vi "UnscentedKalmanFilter_Correct_FuncGroup.vi"(0 "addFuncXExtra":variant, 3 "H_Func":T2, 4 "AddFuncX":T2, 5 "H_FuncExtra":variant, 6 "residualFuncXExtra":variant, 7 "MeanFuncY":T2, 8 "ResidualFuncX":T2, 9 "residualFuncYExtra":variant, 10 "ResidualFuncY":T2, 11 "MeanFuncYExtra":variant) -> (1 "Error":errorcluster, 2 "UNSCENTED_KALMAN_CORRECT_FUNC_GROUP":T1)   [LabVIEW 2019, in "Trajectory_Library.lvlib"]
doc: "Creates a new packed function group cluster to pass to the Correct subVI.\n \nInputs:\n - H_Func -- A vector-valued function of x and u that returns the measurement vector.\n - H_ExtraData -- Variant containing extra data used by the H function. The contents of the variant are specific to the H function.\n - meanFuncY -- A strict function reference that computes the mean of 2 States + 1 measurement vectors using a given set of weights.\n - meanFuncYExtra -- Variant containing extra data used by the meanY function. The contents of the variant are specific to the function.\n - residualFuncY -- A strict function reference that computes the residual of two measurement vectors (i.e. it subtracts them.)\n - residualFuncYExtra -- Variant containing extra data used by the residualY function. The contents of the variant are specific to the function.\n - residualFuncX -- A strict function reference that computes the residual of two state vectors (i.e. it subtracts them.)\n - residualFuncXExtra -- Variant containing extra data used by the residualX function. The contents of the variant are specific to the function.\n - addFuncX -- A strict function reference that adds two state vectors.\n - addFuncXExtra -- Variant containing extra data used by the addY function. The contents of the variant are specific to the function.\n\nOutputs:\n - UnscentedKalmanFilterCorrectFuncGroup -- Cluster containing the functions and extra data.\n - Error -- If TRUE, an error occured."
uses:
  Trajectory_Library.lvlib
  TypeDef/CALLBACK_FUNC_TYPE.ctl
  TypeDef/UNSCENTED_KALMAN_CORRECT_FUNC_GROUP.ctl
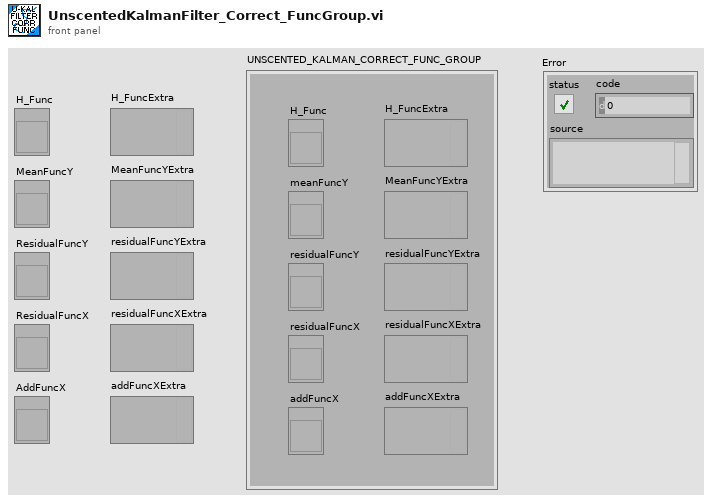
[diagram p1: front panel]
types:
  T1 = typedef "Trajectory_Library.lvlib/UNSCENTED_KALMAN_CORRECT_FUNC_GROUP.ctl" = cluster{"H_Func":T2, "meanFuncY":T2, "residualFuncY":T2, "residualFuncX":T2, "addFuncX":T2, "H_FuncExtra":variant, "MeanFuncYExtra":variant, "residualFuncYExtra":variant, "residualFuncXExtra":variant, "addFuncXExtra":variant}
  T2 = typedef "Trajectory_Library.lvlib/CALLBACK_FUNC_TYPE.ctl" = refnum<vi>
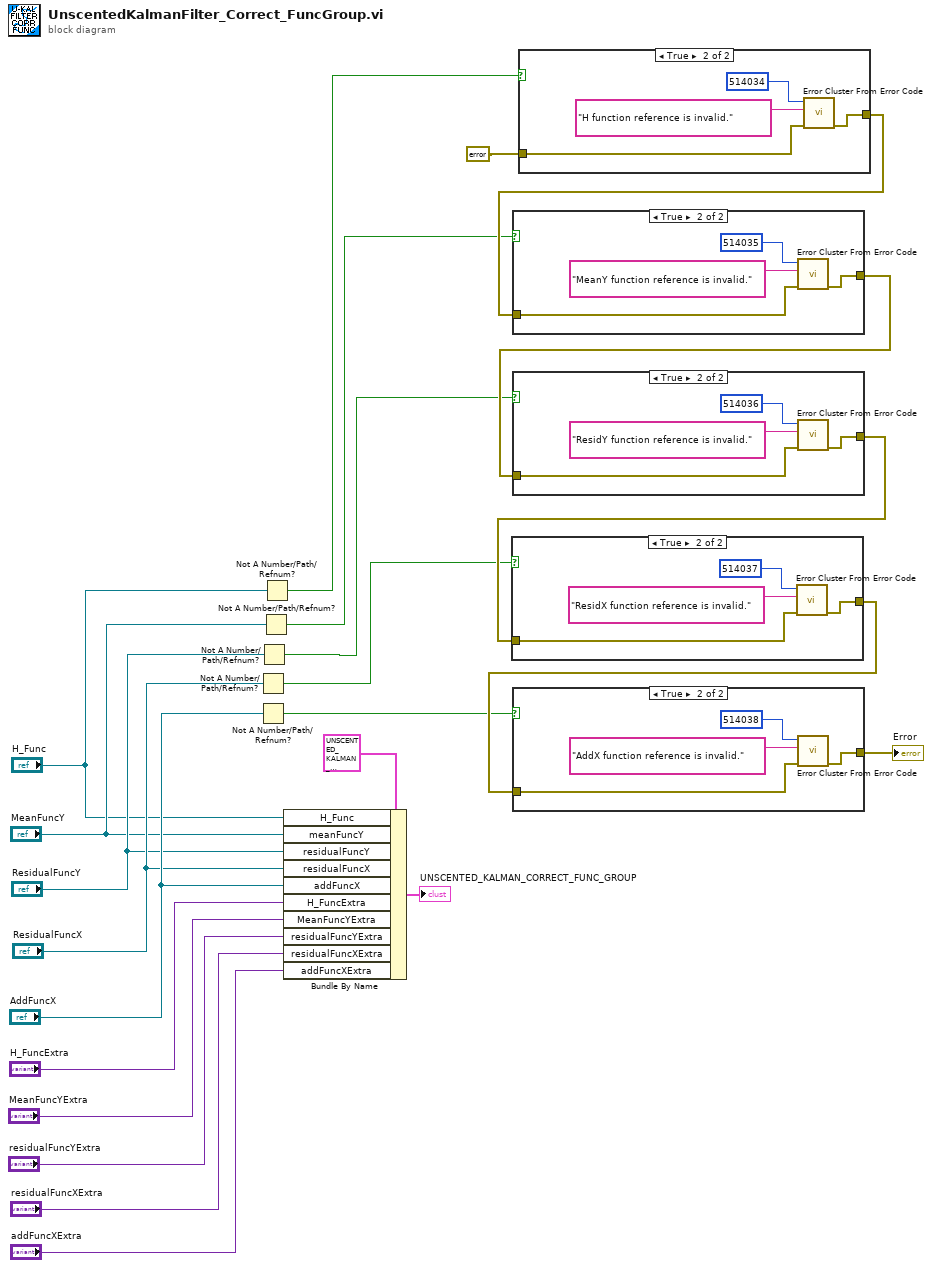
[diagram p0: block diagram]
diagram:
  n1 = Not A Number/Path/Refnum?(number/path/refnum="ResidualFuncX") -> (NaN/Path/Refnum?=w3:bool)
  n2 = Not A Number/Path/Refnum?(number/path/refnum="AddFuncX") -> (NaN/Path/Refnum?=w2:bool)
  n3 = Not A Number/Path/Refnum?(number/path/refnum="ResidualFuncY") -> (NaN/Path/Refnum?=w4:bool)
  n4 = Not A Number/Path/Refnum?(number/path/refnum="MeanFuncY") -> (NaN/Path/Refnum?=w5:bool)
  n5 = Not A Number/Path/Refnum?(number/path/refnum="H_Func") -> (NaN/Path/Refnum?=w6:bool)
  n6 = Bundle By Name(cluster=T1 {"H_Func"=refnum, "meanFuncY"=refnum, "residualFuncY"=refnum, "residualFuncX"=refnum, "addFuncX"=refnum, "H_FuncExtra"=variant, "MeanFuncYExtra"=variant, "residualFuncYExtra"=variant, "residualFuncXExtra"=variant, "addFuncXExtra"=variant} ("UNSCENTED_KALMAN_FILTER_FUNC_GROUP"), "H_Func"="H_Func", "meanFuncY"="MeanFuncY", "residualFuncY"="ResidualFuncY", "residualFuncX"="ResidualFuncX", "addFuncX"="AddFuncX", "H_FuncExtra"="H_FuncExtra", "MeanFuncYExtra"="MeanFuncYExtra", "residualFuncYExtra"="residualFuncYExtra", "residualFuncXExtra"="residualFuncXExtra", "addFuncXExtra"="addFuncXExtra") -> (→"UNSCENTED_KALMAN_CORRECT_FUNC_GROUP":T1)
  n7 = case shown="True" w6 {
    tunnel: errorcluster {"status"=FALSE, "code"=0, "source"=""} ("error constant") -> [w24 w27]
    tunnel: [w24 w28] -> w10
    frame False {
    }
    frame True {
      n8 = call <vilib>:"Error Cluster From Error Code.vi"("error in (no error)"=w27, "error message (\"\")"="H function reference is invalid." ("error message (\"\")"), "error code (0)"=514034) -> ("error out"=w28:errorcluster)  [unwired: 6 in]
    }
  }
  n9 = case shown="True" w5 {
    tunnel: w10 -> [w29 w32]
    tunnel: [w29 w33] -> w9
    frame False {
    }
    frame True {
      n10 = call <vilib>:"Error Cluster From Error Code.vi"("error in (no error)"=w32, "error message (\"\")"="MeanY function reference is invalid." ("error message (\"\")"), "error code (0)"=514035) -> ("error out"=w33:errorcluster)  [unwired: 6 in]
    }
  }
  n11 = case shown="True" w4 {
    tunnel: w9 -> [w34 w37]
    tunnel: [w34 w38] -> w8
    frame False {
    }
    frame True {
      n12 = call <vilib>:"Error Cluster From Error Code.vi"("error in (no error)"=w37, "error message (\"\")"="ResidY function reference is invalid." ("error message (\"\")"), "error code (0)"=514036) -> ("error out"=w38:errorcluster)  [unwired: 6 in]
    }
  }
  n13 = case shown="True" w3 {
    tunnel: w8 -> [w39 w42]
    tunnel: [w39 w43] -> w7
    frame False {
    }
    frame True {
      n14 = call <vilib>:"Error Cluster From Error Code.vi"("error in (no error)"=w42, "error message (\"\")"="ResidX function reference is invalid." ("error message (\"\")"), "error code (0)"=514037) -> ("error out"=w43:errorcluster)  [unwired: 6 in]
    }
  }
  n15 = case shown="True" w2 {
    tunnel: w7 -> [w44 w47]
    tunnel: [w44 w48] -> w1
    frame False {
    }
    frame True {
      n16 = call <vilib>:"Error Cluster From Error Code.vi"("error in (no error)"=w47, "error message (\"\")"="AddX function reference is invalid." ("error message (\"\")"), "error code (0)"=514038) -> ("error out"=w48:errorcluster)  [unwired: 6 in]
    }
  }
  "Error" <- w1
